vi "Unregister Handler.vi"(6 "stop notifier":refnum<notifier>, 8 "response notifier":refnum<notifier>, 9 "handler name":string, 10 "indicator data in":refnum<data-value>, 11 "registry in":T1[](array[typedef])) -> (2 "indicator data out":refnum<data-value>, 3 "registry out":T1[](array[typedef]))   [LabVIEW 2018, in "GLog.lvlib" / "UI Updater.lvlib"]
uses:
  UI Updater.lvlib
  Indicator Data.ctl
  Handler Registration.ctl
  Unregister Response Data.ctl
  f2c0042a-8e76-4380-85f2-45fd47606325.vi
panel:
  # "Connector Pane"
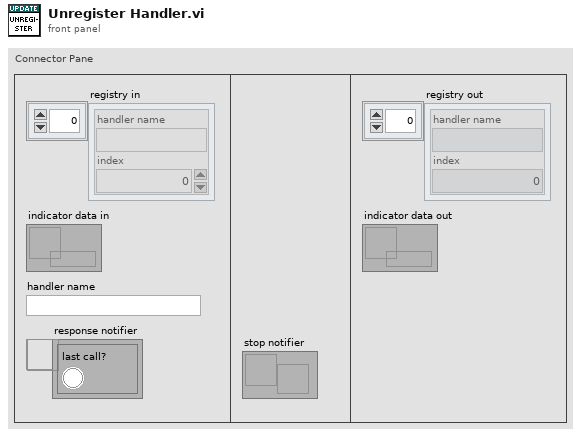
[diagram p1: front panel]
types:
  T1 = typedef "GLog.lvlib/UI Updater.lvlib/Handler Registration.ctl" = cluster{"handler name":string, "index":i32}
  T2 = typedef "GLog.lvlib/UI Updater.lvlib/Unregister Response Data.ctl" = cluster{"last call?":bool}
  T3 = typedef "GLog.lvlib/UI Updater.lvlib/Indicator Data.ctl" = cluster{"Ctl Ref":refnum<vi>, "Log Buffer":string[], "Log Limit":i32, "Line Limit":i32, "Autoscroll?":bool, "Valid?":bool, "Owning VI":refnum<vi>, "Ctl Index":i32, "Needs Write?":bool}
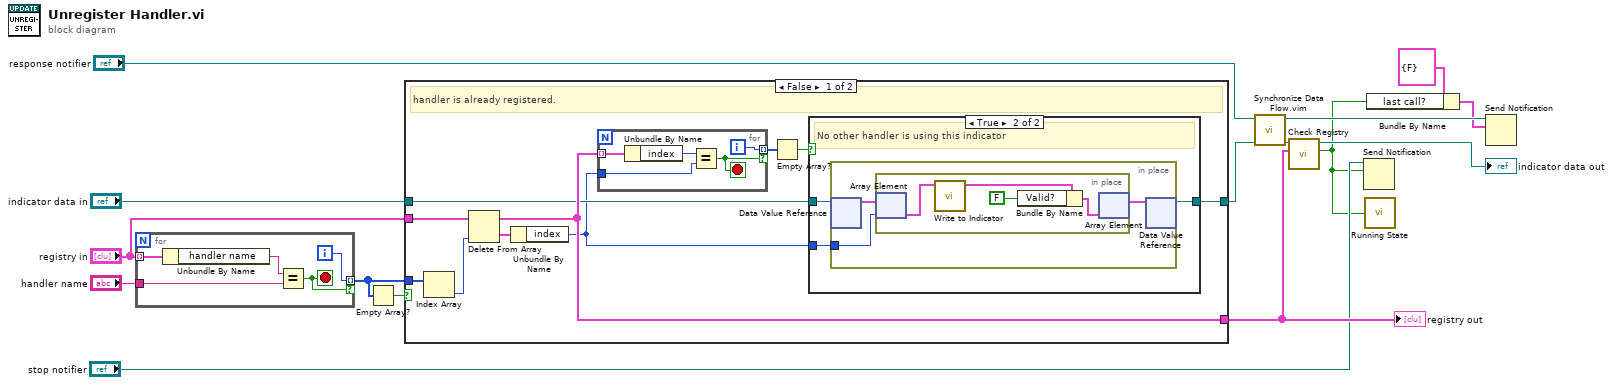
[diagram p0: block diagram]
diagram:
  n1 = for {
    tunnel: "registry in" -> [w20] mode=indexing
    tunnel: "handler name" -> [w19]
    tunnel: [w17] -> w13 mode=indexing if=w16
    i -> [w17]
    stop <- w16 stop-if-true
    n2 = Unbundle By Name(w20) -> ("handler name"=w18:string)
    n3 = Equal?(x=w18, y=w19) -> (x = y?=w16:bool)
  }
  n4 = Empty Array?(array=w13) -> (empty?=w12:bool)
  n5 = case shown="False" w12 {
    tunnel: w13 -> [w30 _]
    tunnel: "registry in" -> [w28 w48]
    tunnel: [w26 w48] -> w3
    tunnel: "indicator data in" -> [w23 w47]
    tunnel: [w22 w47] -> w10
    frame False {
      # "handler is already registered."
      n6 = Index Array(array=w30) -> (element=w29:i32)  [unwired: 1 in]
      n7 = Delete From Array(array=w28, index=w29) -> (deleted portion=w27:T1, array with subset deleted=w26:T1[])  [unwired: 1 in]
      n8 = Unbundle By Name(w27) -> ("index"=w21:i32)
      n9 = for {
        tunnel: w26 -> [w46] mode=indexing
        tunnel: w21 -> [w45]
        tunnel: [w43] -> w25 mode=indexing if=w42
        i -> [w43]
        stop <- w42 stop-if-true
        n10 = Unbundle By Name(w46) -> ("index"=w44:i32)
        n11 = Equal?(x=w44, y=w45) -> (x = y?=w42:bool)
      }
      n12 = Empty Array?(array=w25) -> (empty?=w24:bool)
      n13 = case shown="True" w24 {
        tunnel: w23 -> [w31 w34]
        tunnel: [w31 w33] -> w22
        tunnel: w21 -> [_ w32]
        frame False {
          # "Another handler is still using this indicator."
        }
        frame True {
          # "No other handler is using this indicator"
          n14 = in-place {
            in-place-border: w32 -> [w36]
            n15 = in-place-dvr #1(w34) -> (w37:T3[])  [unwired: 1 out]
            n16 = in-place {
              n17 = in-place-array #2(w37, w36) -> (w39:T3)
              n18 = call "Write to Indicator.vi"("indicator data in"=w39) -> ("indicator data out"=w38:T3)  [unwired: 9 in, 1 out]
              n19 = Bundle By Name(cluster=w38, "Valid?"=FALSE) -> (w40:T3)
              n20 = in-place-array #2(w40) -> (w35:T3[])  [unwired: 1 out]
            }
            n21 = in-place-dvr #1(w35) -> (w33:refnum<data-value>)  [unwired: 1 out]
          }
        }
      }
    }
    frame True {
      # "handler is not registered"
    }
  }
  "registry out" <- w3
  n22 = call "Synchronize Data Flow.vim"("input 4"=w10, "input 1"="response notifier") -> ("output 4"=w8:refnum<data-value>, "output 1"=w6:refnum<notifier>)  [unwired: 2 in, 2 out]
  n23 = call "Check Registry.vi"("registry"=w3, "indicator data in"=w8) -> ("empty registry?"=w1:bool, "indicator data out"=→"indicator data out":refnum<data-value>)  [unwired: 8 in]
  n24 = Send Notification(notification=w1, notifier="stop notifier") -> ()  [unwired: 1 in, 2 out]
  n25 = call "Running State.vi"("Reset? (F)"=w1) -> ()  [unwired: 1 out]
  n26 = Bundle By Name(cluster=T2 {"last call?"=FALSE} ("unregister response data"), "last call?"=w1) -> (w4:T2)
  n27 = Send Notification(notification=w4, notifier=w6) -> ()  [unwired: 1 in, 2 out]
